vi "Get TDF File List.vi"(8 "error in (no error)":errorcluster caption="에러 입력(에러 없음)", 11 "Instrument Manager 입력":refnum<class "Instrument Manager.lvclass">) -> (0 "error out":errorcluster caption="에러 출력", 2 "File List":string[](array[string]), 3 "Instrument Manager 출력":refnum<class "Instrument Manager.lvclass">)   [LabVIEW 2023, in "Instrument Manager.lvclass"]
uses:
  Instrument Manager.lvclass
  Instrument Manager.lvclass/Instrument Manager.ctl
  Module/Spectrum Analyzer/Interface_Spectrum/Interface_Spectrum.lvclass
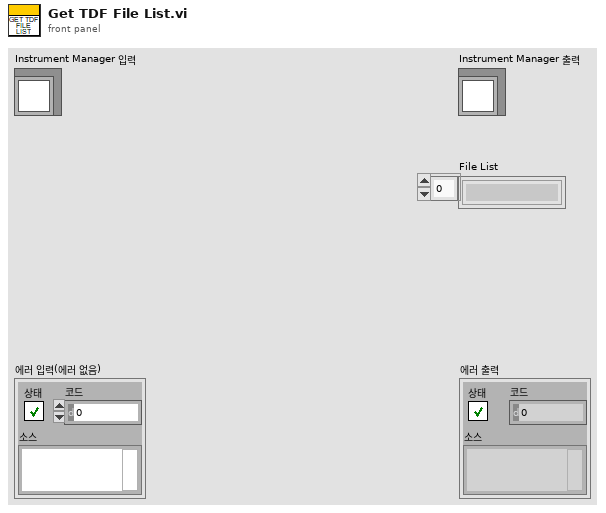
[diagram p1: front panel]
types:
  T1 = cluster{"Anritsu Call Box":refnum<class "Anritsu Call Box.lvclass">, "Spectrum Analyzer":refnum<class "Interface_Spectrum.lvclass">, "RF Switch Box":refnum<class "RF Filter Box.lvclass">, "Turn Table":refnum<class "Interface - Turn Table.lvclass">, "Mast":refnum<class "Interface - Mast.lvclass">, "3D Controller":refnum<class "Interface_3D Controller.lvclass">}
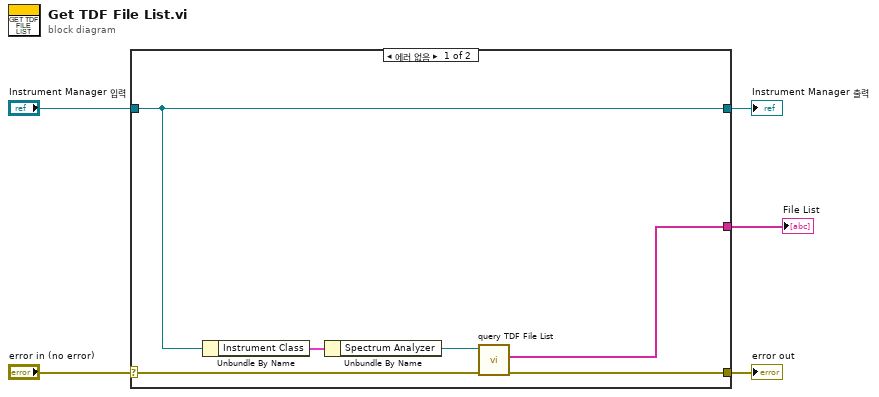
[diagram p0: block diagram]
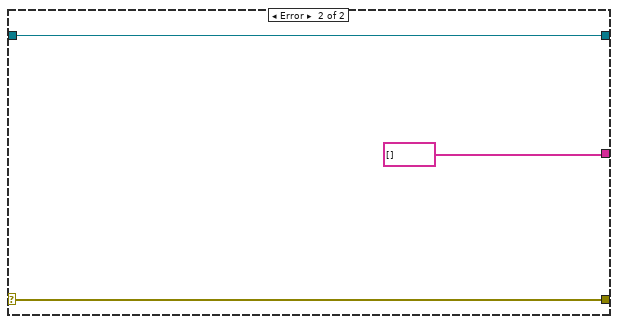
[diagram p2: hidden frame]
diagram:
  n1 = case shown="에러 없음" "error in (no error)" {
    selector: "error in (no error)" -> [w9 w14]
    tunnel: [w7 w14] -> w4
    tunnel: [w11 w13] -> w2
    tunnel: "Instrument Manager 입력" -> [w11 w13]
    tunnel: [w6 string[] [] ("File List")] -> w1
    frame No Error {
      n2 = Unbundle By Name(w11) -> ("Instrument Class"=w10:T1)
      n3 = Unbundle By Name(w10) -> ("Spectrum Analyzer"=w8:refnum<class "Interface_Spectrum.lvclass">)
      n4 = call-dynamic "query TDF File List.vi"("error in (no error)"=w9, "Interface_Spectrum 입력"=w8) -> ("error out"=w7:errorcluster, "File List"=w6:string[])  [unwired: 7 in, 1 out]
    }
    frame Error {
    }
  }
  "error out" <- w4
  "Instrument Manager 출력" <- w2
  "File List" <- w1
